vi "Wait until VIs close.vi"(8 "error in (no error)":errorcluster, 10 "Timeout (s)":dbl=-1.0 format="%#_13g", 11 "VI Ref In[]":refnum<vi>[](array[refnum])) -> (0 "error out":errorcluster, 1 "Unclosed VIs[]":refnum<vi>[](array[refnum]), 2 "Timed Out?":bool, 3 "VIs Ref Out[]":refnum<vi>[](array[refnum]))   [LabVIEW 2016, in "SLL Application.lvlib"]
doc: "Waits for either all VIs wired in the input (as reference) to close, or the specified timeout occurs, whichever is earlier.\nThis VI does not close the reference of the input VIs. This VI runs normally even if an error occurred before this VI."
uses:
  SLL Application.lvlib
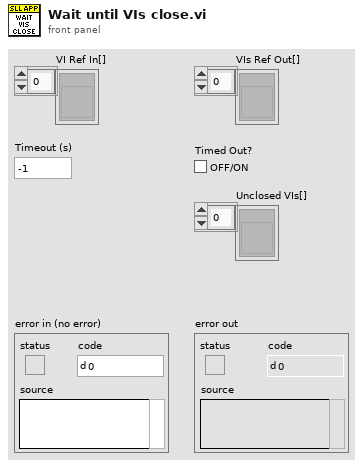
[diagram p1: front panel]
types:
  T1 = enum32{"Bad", "Idle", "Run top level", "Running"}
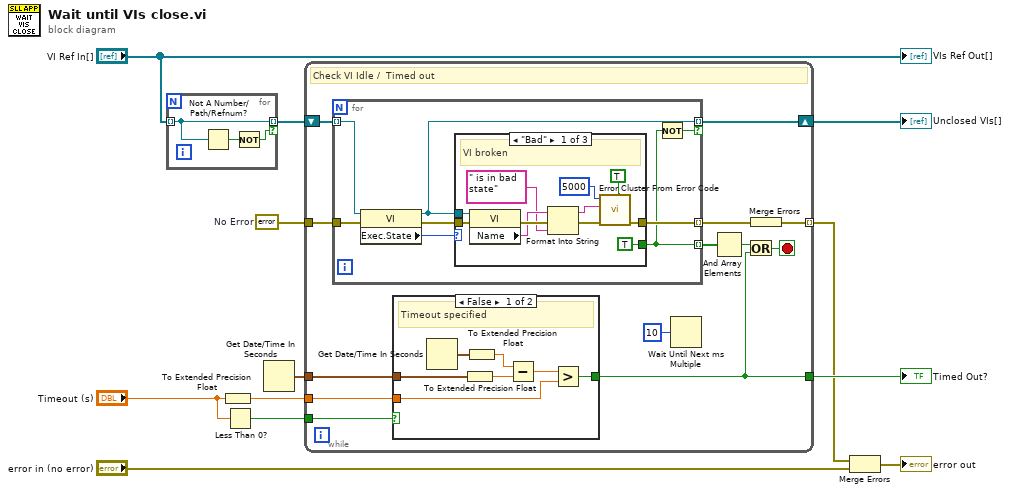
[diagram p0: block diagram]
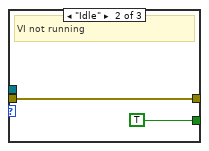
[diagram p2: hidden frame]
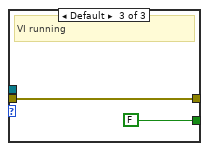
[diagram p3: hidden frame]
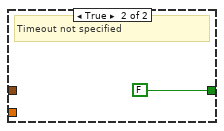
[diagram p4: hidden frame]
diagram:
  w4 = errorcluster {"status"=FALSE, "code"=0, "source"=""}  # No Error
  n1 = for {
    tunnel: "VI Ref In[]" -> [w14] mode=indexing
    tunnel: [w14] -> w3 mode=indexing if=w13
    n2 = Not A Number/Path/Refnum?(number/path/refnum=w14) -> (NaN/Path/Refnum?=w15:bool)
    n3 = Not(x=w15) -> (.not. x?=w13:bool)
  }
  n4 = To Extended Precision Float(1:"Timeout (s)") -> (0:w7:ext)
  n5 = Less Than 0?(x="Timeout (s)") -> (x < 0?=w8:bool)
  n6 = Get Date/Time In Seconds() -> (seconds since 1Jan1904=w5:timestamp)
  n7 = while {
    tunnel: w8 -> [w25]
    tunnel: w7 -> [w24]
    tunnel: [w23] -> w6 mode=indexing
    shift-right: [w26] -> w12
    shift-left: w3 -> [w28]
    tunnel: w5 -> [w22]
    tunnel: w4 -> [w20]
    tunnel: [w18] -> w10
    stop <- w17 stop-if-true
    # "Check VI Idle /  Timed out"
    n8 = for {
      tunnel: w28 -> [w36] mode=indexing
      tunnel: [w35] -> w27 mode=indexing
      tunnel: [w34] -> w26 mode=indexing if=w31
      tunnel: w20 -> [w33]
      tunnel: [w32] -> w19 mode=indexing
      n9 = property class="VI"(reference=w36, error in=w33) -> (reference out=w34:refnum<vi>, error out=w30:errorcluster, "Exec.State"=w29:T1)
      n10 = case shown="\"Bad\"" w29 {
        tunnel: [TRUE TRUE FALSE] -> w32
        tunnel: [w47 w48 w50] -> w35
        tunnel: w30 -> [w42 w48 w50]
        tunnel: w34 -> [w43 _ _]
        frame "Bad" {
          # "VI broken"
          n11 = property class="VI"(reference=w43, error in=w42) -> (error out=w41:errorcluster, "Name"=w39:string)  [unwired: 1 out]
          n12 = Format Into String(initial string=w39, error in=w41, " is in bad state" ("error message (\"\")")) -> (resulting string=w37:string, error out=w40:errorcluster)  [unwired: 1 in]
          n13 = call <vilib>:"Error Cluster From Error Code.vi"("is warning? (False)"=TRUE, "error in (no error)"=w40, "error message (\"\")"=w37, "error code (0)"=5000) -> ("error out"=w47:errorcluster)  [unwired: 5 in]
        }
        frame "Idle" {
          # "VI not running"
        }
        frame Default {
          # "VI running"
        }
      }
      n14 = Not(x=w32) -> (.not. x?=w31:bool)
    }
    n15 = case shown="False" w25 {
      tunnel: w24 -> [w58 _]
      tunnel: w22 -> [w57 _]
      tunnel: [w52 FALSE] -> w18
      frame False {
        # "Timeout specified"
        n16 = Get Date/Time In Seconds() -> (seconds since 1Jan1904=w56:timestamp)
        n17 = To Extended Precision Float(1:w57) -> (0:w55:ext)
        n18 = To Extended Precision Float(1:w56) -> (0:w54:ext)
        n19 = Subtract(x=w54, y=w55) -> (x-y=w53:ext)
        n20 = Greater?(x=w53, y=w58) -> (0:w52:bool)
      }
      frame True {
        # "Timeout not specified"
      }
    }
    n21 = Wait Until Next ms Multiple(millisecond multiple=u32 10) -> ()  [unwired: 1 out]
    n22 = And Array Elements(Boolean array=w19) -> (logical AND=w16:bool)
    n23 = Or(x=w16, y=w18) -> (x .or. y?=w17:bool)
    n24 = Merge Errors(w27) -> (w23:errorcluster)
  }
  "Unclosed VIs[]" <- w12
  "Timed Out?" <- w10
  n25 = Merge Errors(w6, "error in (no error)") -> (→"error out":errorcluster)
  "VIs Ref Out[]" <- "VI Ref In[]"
